vi "KalmanFilter_GetK_Single.vi"(9 "Column":i32, 10 "Row":i32, 11 "in KalmanFilter":T1) -> (0 "Error":bool, 3 "K":dbl)   [LabVIEW 2019, in "Trajectory_Library.lvlib"]
doc: "Returns an element of the steady-state Kalman gain matrix K.\n \nInputs:\n - KalmanFilter -- filter data cluster\n - row -- matrix row indiex (0-n)\n - column -- matrix column index (0-n)\n\nOutputs:\n - K - The steady-state Kalman gain matrix K.\n - Error -- value is TRUE if an error occured."
uses:
  Trajectory_Library.lvlib
  <vilib>/Analysis/Matrix/Datatypes/RealMatrix.ctl
  <vilib>/Analysis/Matrix/NI_Matrix.lvlib
  TypeDef/LINEAR_SYSTEM.ctl
  TypeDef/KALMAN_FILTER.ctl
panel:
  # "Steady State Gain  \n<States,Outputs>"
  # "State Estimate <Statess,1>"
  # "<States,States>"
  # "<States,Inputs>"
  # "<Outputs,States>"
  # "<Outputs,Inputs>"
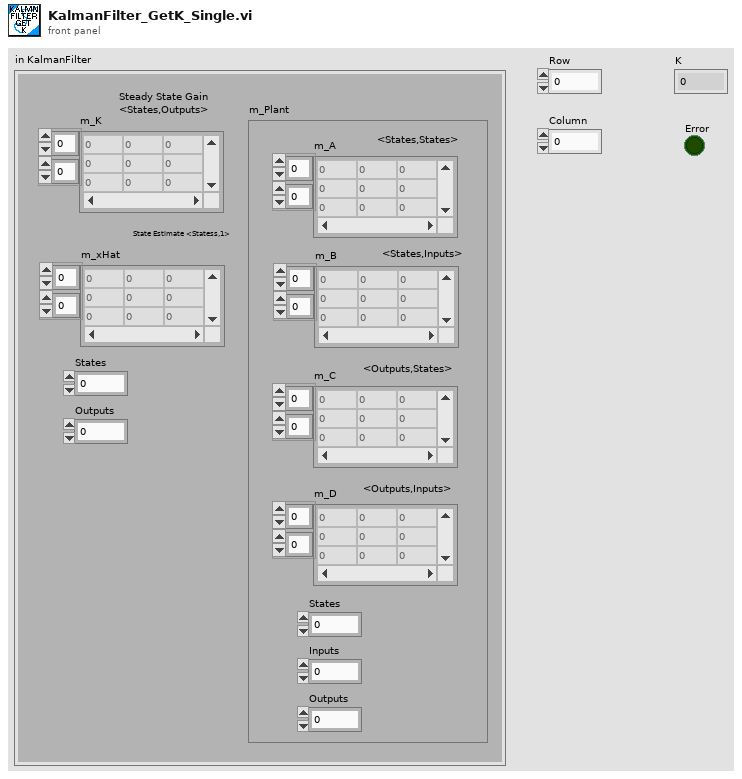
[diagram p1: front panel]
types:
  T1 = typedef "Trajectory_Library.lvlib/KALMAN_FILTER.ctl" = cluster{"m_K":T2, "m_xHat":T2, "States":i32, "Outputs":i32, "m_Plant":T3}
  T2 = typedef "NI_Matrix.lvlib/RealMatrix.ctl" = dbl[][]
  T3 = typedef "Trajectory_Library.lvlib/LINEAR_SYSTEM.ctl" = cluster{"m_A":T2, "m_B":T2, "m_C":T2, "m_D":T2, "States":i32, "Inputs":i32, "Outputs":i32}
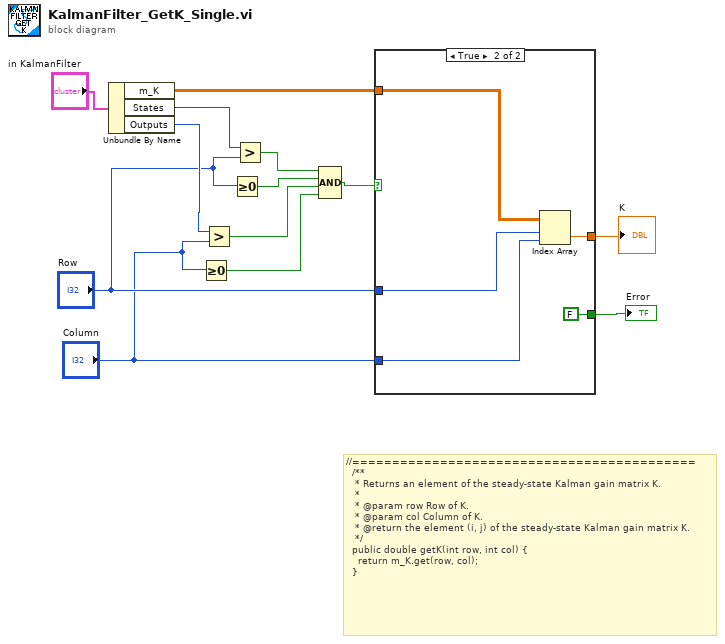
[diagram p0: block diagram]
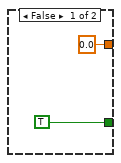
[diagram p2: hidden frame]
diagram:
  # "//===========================================\n  /**\n   * Returns an element of the steady-state Kalman gain matrix K.\n   *\n   * @param row Row of K.\n   * @param col Column of K.\n   * @return the element (i, j) of the steady-state Kalman gain matrix K.\n   */\n  public double getK(int row, int col) {\n    return m_K.get(row, col);\n  }"
  n1 = Unbundle By Name("in KalmanFilter") -> ("m_K"=w12:T2, "States"=w10:i32, "Outputs"=w9:i32)
  n2 = Greater Or Equal To 0?(x="Column") -> (x >= 0?=w3:bool)
  n3 = Greater?(x=w9, y="Column") -> (0:w4:bool)
  n4 = Greater Or Equal To 0?(x="Row") -> (x >= 0?=w5:bool)
  n5 = Greater?(x=w10, y="Row") -> (0:w6:bool)
  n6 = Compound Arithmetic op=AND(w6, w5, w4, w3) -> (w2:bool)
  n7 = case shown="True" w2 {
    tunnel: w12 -> [_ w20]
    tunnel: [0.0 ("Real Matrix Element") w19] -> w11
    tunnel: "Row" -> [_ w18]
    tunnel: "Column" -> [_ w17]
    tunnel: [TRUE FALSE] -> w1
    frame False {
    }
    frame True {
      n8 = Index Array(array=w20, index (row)=w18, index (col)=w17) -> (element=w19:dbl)
    }
  }
  "K" <- w11
  "Error" <- w1
